vi "Get Statistics.vi"(6 "timeout (ms)":i32=5000, 8 "error in":errorcluster, 11 "gRPC ID":T2) -> (0 "error out":errorcluster, 2 "Statistics":T1, 3 "gRPC ID out":T2)   [LabVIEW 2021, in "CAN_Writer_NIXNET_Wrapper.lvlib"]
uses:
  CAN_Writer_NIXNET_Wrapper.lvlib
  <vilib>/gRPC/LabVIEW gRPC Library/Shared/grpcId.ctl
  CanWriterNixnet_client/RPC Messages/cif_can_writer_nixnet_Statistics.ctl
  CanWriterNixnet_client/CanWriterNixnet_client.lvlib
  <vilib>/gRPC/LabVIEW gRPC Library/grpc-lvsupport-release.lvlib
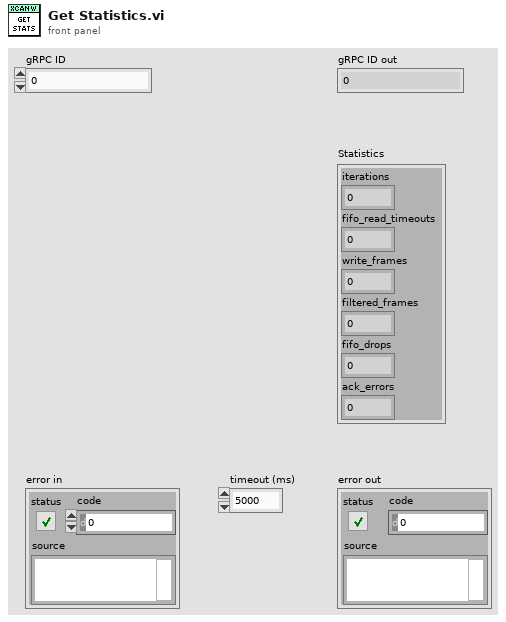
[diagram p1: front panel]
types:
  T1 = typedef "CanWriterNixnet_client.lvlib/cif_can_writer_nixnet_Statistics.ctl" = cluster{"iterations":u64, "fifo_read_timeouts":u64, "write_frames":u64, "filtered_frames":u64, "fifo_drops":u64, "ack_errors":u64}
  T2 = typedef "grpc-lvsupport-release.lvlib/grpcId.ctl" = u64
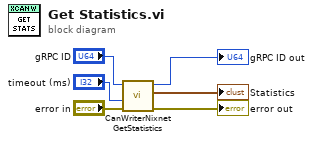
[diagram p0: block diagram]
diagram:
  n1 = call "CanWriterNixnet GetStatistics.vi"("error in"="error in", "timeout (ms)"="timeout (ms)", "gRPC ID"="gRPC ID") -> ("error out"=→"error out":errorcluster, "Response Data"=→"Statistics":T1, "gRPC ID out"=→"gRPC ID out":T2)  [unwired: 6 in]
